vi "Own20261012_SetForStopIfTrue.vi"() -> ()   [LabVIEW 2024]
panel:
  out "error out":errorcluster caption="错误输出"
  in  "stop_if_true":bool
  in  "for_id":u32
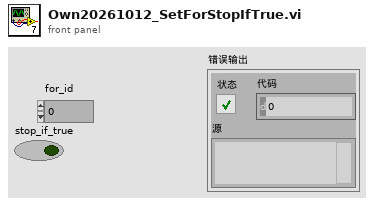
[diagram p1: front panel]
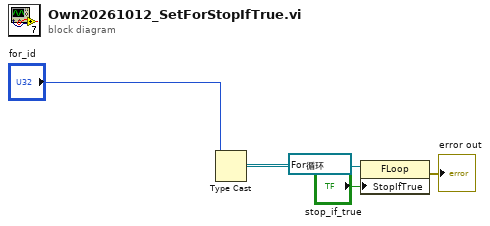
[diagram p0: block diagram]
diagram:
  n1 = Type Cast(type=refnum<vi> refnum ("引用"), x="for_id") -> (*(type *) &x=w3:refnum<vi>)
  n2 = property class="FLoop"(reference=w3, "StopIfTrue"="stop_if_true") -> (error out=→"error out":errorcluster)  [unwired: 1 in, 1 out]
